vi "work2_Cooker_Module.vi"() -> ()   [LabVIEW 2026]
panel:
  in  "Numeric":dbl
  in  "Burgers":bool
  in  "Meal":bool
  in  "stop":bool
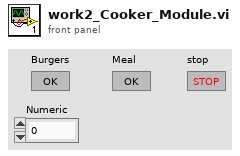
[diagram p1: front panel]
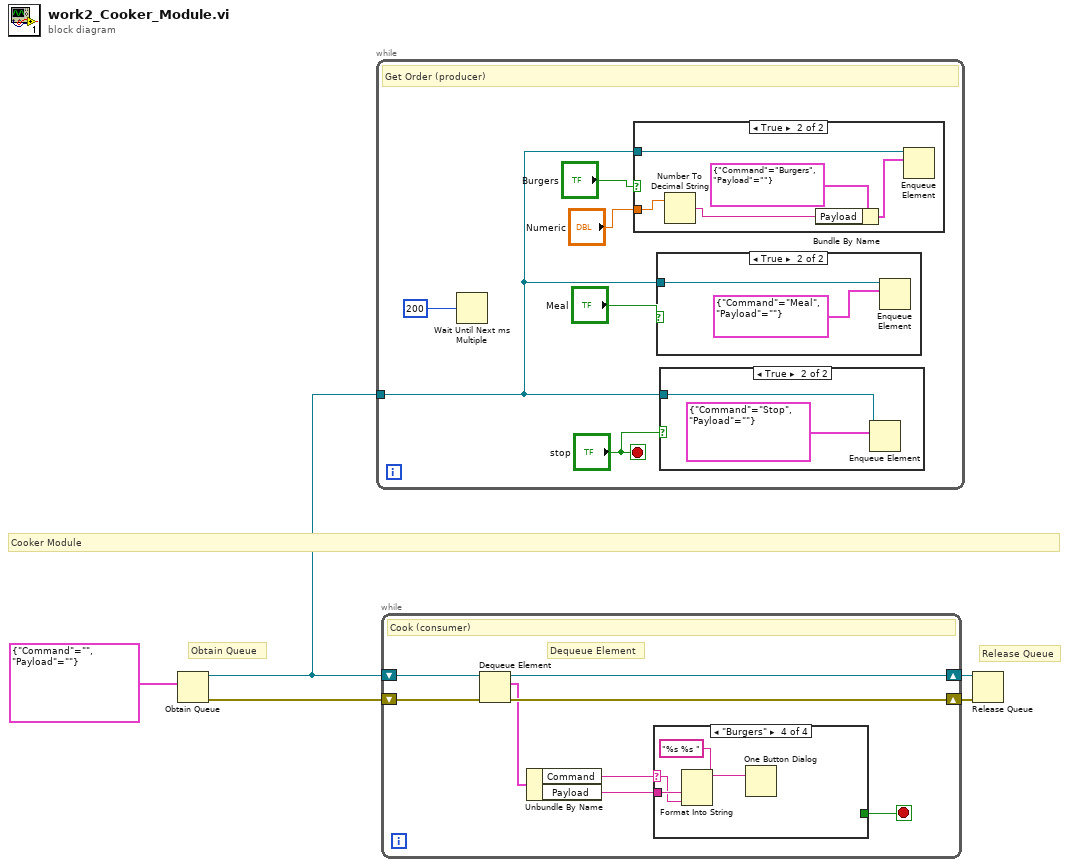
[diagram p0: block diagram]
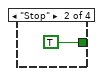
[diagram p6: hidden frame]
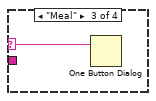
[diagram p7: hidden frame]
diagram:
  # "Cooker Module"
  # "Release Queue"
  # "Obtain Queue"
  n1 = Obtain Queue(element data type=cluster{"Command":string, "Payload":string} {"Command"="", "Payload"=""}) -> (queue out=w2:refnum<queue>, error out=w5:errorcluster)  [unwired: 4 in, 1 out]
  n2 = while {
    tunnel: w2 -> [w7]
    stop <- "stop" stop-if-true
    # "Get Order (producer)"
    n3 = Wait Until Next ms Multiple(millisecond multiple=u32 200) -> ()  [unwired: 1 out]
    n4 = case shown="True" "Burgers" {
      tunnel: w7 -> [_ w16]
      tunnel: "Numeric" -> [_ w13]
      frame False {
      }
      frame True {
        n5 = Number To Decimal String(number=w13) -> (decimal integer string=w12:string)  [unwired: 1 in]
        n6 = Bundle By Name(cluster=cluster{"Command":string, "Payload":string} {"Command"="Burgers", "Payload"=""} ("element"), "Payload"=w12) -> (w14:cluster{"Command":string, "Payload":string})
        n7 = Enqueue Element(queue=w16, element=w14) -> ()  [unwired: 2 in, 3 out]
      }
    }
    n8 = case shown="True" "Meal" {
      tunnel: w7 -> [_ w18]
      frame False {
      }
      frame True {
        n9 = Enqueue Element(queue=w18, element=cluster{"Command":string, "Payload":string} {"Command"="Meal", "Payload"=""}) -> ()  [unwired: 2 in, 3 out]
      }
    }
    n10 = case shown="True" "stop" {
      tunnel: w7 -> [_ w20]
      frame False {
      }
      frame True {
        n11 = Enqueue Element(queue=w20, element=cluster{"Command":string, "Payload":string} {"Command"="Stop", "Payload"=""}) -> ()  [unwired: 2 in, 3 out]
      }
    }
  }
  n12 = while {
    shift-right: [w26] -> w3
    shift-left: w5 -> [w28]
    shift-right: [w27] -> w4
    shift-left: w2 -> [w25]
    stop <- w22 stop-if-true
    # "Dequeue Element"
    # "Cook (consumer)"
    n13 = Dequeue Element(queue=w25, error in (no error)=w28) -> (queue out=w27:refnum<queue>, element=w24:cluster{"Command":string, "Payload":string}, error out=w26:errorcluster)  [unwired: 1 in, 1 out]
    n14 = Unbundle By Name(w24) -> ("Command"=w23:string, "Payload"=w21:string)
    n15 = case shown="\"Burgers\"" w23 {
      selector: w23 -> [_ _ w30 w31]
      tunnel: [_ TRUE _ _] -> w22
      tunnel: w21 -> [_ _ _ w32]
      frame Default {
      }
      frame "Stop" {
      }
      frame "Meal" {
        n16 = One Button Dialog(message=w30) -> ()  [unwired: 1 in, 1 out]
      }
      frame "Burgers" {
        n17 = Format Into String(format string="%s %s ", w32, w31) -> (resulting string=w33:string)  [unwired: 2 in, 1 out]
        n18 = One Button Dialog(message=w33) -> ()  [unwired: 1 in, 1 out]
      }
    }
  }
  n19 = Release Queue(queue=w4, error in (no error)=w3) -> ()  [unwired: 1 in, 3 out]
